vi "init.vi"(8 "error in (no error)":errorcluster, 9 "certificatePath":string, 10 "address":string="127.0.0.1:50051", 11 "rotationTable in":refnum<class "rotationTable.lvclass">) -> (0 "error out":errorcluster, 3 "rotationTable out":refnum<class "rotationTable.lvclass">)   [LabVIEW 2020, in "rotationTable.lvclass"]
uses:
  rotationTable.lvclass
  <vilib>/gRPC/LabVIEW gRPC Library/Shared/grpcId.ctl
  lexitekDriver_client/RPC Messages/frontend_message.ctl
  rotationTable.lvclass/rotationTable.ctl
  lexitekDriver_client/lexitekDriver_client.lvlib
  <vilib>/gRPC/LabVIEW gRPC Library/grpc-lvsupport-release.lvlib
panel:
  in  "RUN":T1={"source"="lvClient::init", "command"="RUN=1500", "timestamp_ms"=0}
  in  "CALIBRATE":T1={"source"="lvClient::init", "command"="CALIBRATE", "timestamp_ms"=0}
  out "gRPC ID Out":T2
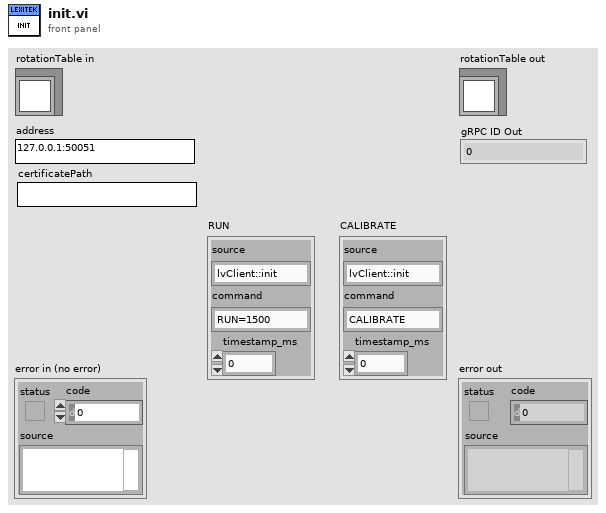
[diagram p1: front panel]
types:
  T1 = typedef "lexitekDriver_client.lvlib/frontend_message.ctl" = cluster{"source":string, "command":string, "timestamp_ms":u64}
  T2 = typedef "grpc-lvsupport-release.lvlib/grpcId.ctl" = u64
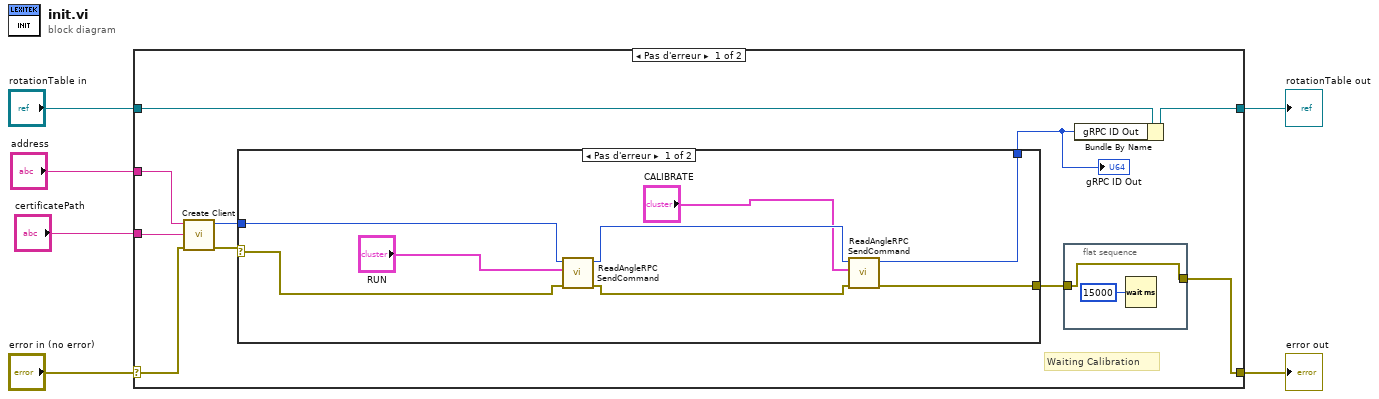
[diagram p0: block diagram]
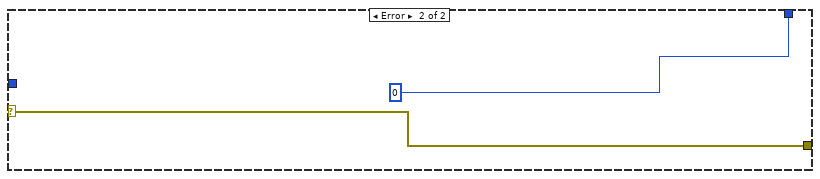
[diagram p2: hidden frame]
diagram:
  n1 = case shown="Pas d'erreur" "error in (no error)" {
    selector: "error in (no error)" -> [w16 w30]
    tunnel: [w7 w30] -> w5
    tunnel: [w13 w29] -> w3
    tunnel: "rotationTable in" -> [w12 w29]
    tunnel: "address" -> [w15 _]
    tunnel: "certificatePath" -> [w14 _]
    frame No Error {
      # "Waiting Calibration"
      n2 = call "Create Client.vi"("error in"=w16, "certificatePath"=w14, "address"=w15) -> ("error out"=w11:errorcluster, "gRPC ID Out"=w10:T2)  [unwired: 7 in]
      n3 = case shown="Pas d'erreur" w11 {
        selector: w11 -> [w21 w27]
        tunnel: w10 -> [w23 _]
        tunnel: [w26 T2 0 ("gRPC ID Out")] -> w9
        tunnel: [w25 w27] -> w8
        frame No Error {
          n4 = call "ReadAngleRPC SendCommand.vi"("error in"=w21, "Request Data"="RUN", "gRPC ID"=w23) -> ("error out"=w24:errorcluster, "gRPC ID out"=w22:T2)  [unwired: 6 in, 1 out]
          n5 = call "ReadAngleRPC SendCommand.vi"("error in"=w24, "Request Data"="CALIBRATE", "gRPC ID"=w22) -> ("error out"=w25:errorcluster, "gRPC ID out"=w26:T2)  [unwired: 6 in, 1 out]
        }
        frame Error {
        }
      }
      "gRPC ID Out" <- w9
      n6 = flat-sequence {
        tunnel: [w17] -> w7
        tunnel: w8 -> [w17]
        frame #0 {
          n7 = Wait (ms)(milliseconds to wait=u32 15000 ("attente (ms)")) -> ()  [unwired: 1 out]
        }
      }
      n8 = Bundle By Name(cluster=w12, "gRPC ID Out"=w9) -> (w13:refnum<class "rotationTable.lvclass">)
    }
    frame Error {
    }
  }
  "error out" <- w5
  "rotationTable out" <- w3
